vi "Remove Default Error Description.vi"(11 "description":string) -> (3 "description out":string)   [LabVIEW 2020, in "MCP Server.lvlib"]
doc: "Returns description unchanged, or an empty string when it is one of LabVIEW's default descriptions of an error cluster: the help text of NI's error in and error out controls (vi.lib\\errclust.llb, the same in LabVIEW 2020 and 2026) or of their status, code and source elements. tools/list leaves an empty description out, so that help text, written for the front panel, does not reach the MCP client, while a description the tool's author wrote is kept.\n\nBefore comparing, CR LF and CR become LF and white space at the start and end is removed. Otherwise the text has to match exactly: a description that only begins with NI's wording is the author's and is kept."
uses:
  MCP Server.lvlib
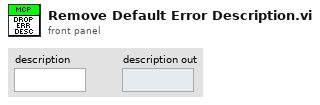
[diagram p1: front panel]
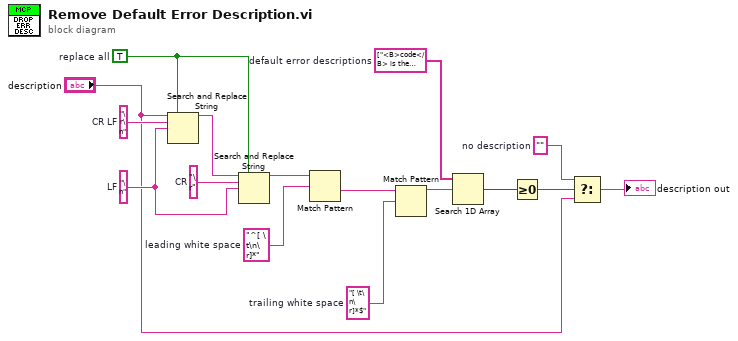
[diagram p0: block diagram]
diagram:
  w4 = ""  # no description
  w7 = string[] ["<B>code</B> is the error or warning code.\n\nRight-click the <B>error in</B> control on the front panel and select <B>Explain Error</B> or <B>Explain Warning</B> from the shortcut menu for more information about the error.", "<B>code</B> is the error or warning code.\n\nRight-click the <B>error out</B> indicator on the front panel and select <B>Explain Error</B> or <B>Explain Warning</B> from the shortcut menu for more information about the error.", "<B>error in</B> can accept error information wired from VIs previously called. Use this information to decide if any functionality should be bypassed in the event of errors from other VIs.\n\nRight-click the <B>error in</B> control on the front panel and select <B>Explain Error</B> or <B>Explain Warning</B> from the shortcut menu for more information about the error.", "<B>error out</B> passes error or warning information out of a VI to be used by other VIs.\n\nRight-click the <B>error out</B> indicator on the front panel and select <B>Explain Error</B> or <B>Explain Warning</B> from the shortcut menu for more information about the error.", "<B>source</B> describes the origin of the error or warning.\n\nRight-click the <B>error in</B> control on the front panel and select <B>Explain Error</B> or <B>Explain Warning</B> from the shortcut menu for more information about the error.", "<B>source</B> string describes the origin of the error or warning.\n\nRight-click the <B>error out</B> indicator on the front panel and select <B>Explain Error</B> or <B>Explain Warning</B> from the shortcut menu for more information about the error.", "<B>status</B> is TRUE (X) if an error occurred or FALSE (checkmark) to indicate a warning or that no error occurred.\n\nRight-click the <B>error in</B> control on the front panel and select <B>Explain Error</B> or <B>Explain Warning</B> from the shortcut menu for more information about the error.", "<B>status</B> is TRUE (X) if an error occurred or FALSE (checkmark) to indicate a warning or that no error occurred.\n\nRight-click the <B>error out</B> indicator on the front panel and select <B>Explain Error</B> or <B>Explain Warning</B> from the shortcut menu for more information about the error."]  # default error descriptions
  w8 = "[ \t\n\r]*$"  # trailing white space
  w10 = "^[ \t\n\r]*"  # leading white space
  w12 = TRUE  # replace all
  w13 = "\n"  # LF
  w14 = "\r"  # CR
  w16 = "\r\n"  # CR LF
  n1 = Search and Replace String(replace all?=w12, input string="description", search string=w16, replace string=w13) -> (result string=w15:string)  [unwired: 4 in, 3 out]
  n2 = Search and Replace String(replace all?=w12, input string=w15, search string=w14, replace string=w13) -> (result string=w11:string)  [unwired: 4 in, 3 out]
  n3 = Match Pattern(string=w11, regular expression=w10) -> (after substring=w9:string)  [unwired: 1 in, 3 out]
  n4 = Match Pattern(string=w9, regular expression=w8) -> (before substring=w6:string)  [unwired: 1 in, 3 out]
  n5 = Search 1D Array(1D array=w7, element=w6) -> (index of element=w5:i32)  [unwired: 1 in]
  n6 = Greater Or Equal To 0?(x=w5) -> (x >= 0?=w3:bool)
  n7 = Select(t=w4, s=w3, f="description") -> (s? t:f=→"description out":string)
